vi "Pre Launch Init.vi"(11 "GlobalPlanner in":refnum<class "GlobalPlanner.lvclass"> caption="操作者输入") -> (0 "error out":errorcluster caption="错误输出", 3 "GlobalPlanner out":refnum<class "GlobalPlanner.lvclass"> caption="操作者输出")   [LabVIEW 2014, in "GlobalPlanner.lvlib" / "GlobalPlanner.lvclass"]
doc: "(<B>Filename</B>: Actor Framework.lvlib:Actor.lvclass:Pre Launch Init.vi)\n\nDefines behavior that occurs after the Launch Nested Actor method is invoked but before the actor's Actor Core method begins running.\n\nBy default, this method does nothing. A descendant class may override it to define behavior."
uses:
  GlobalPlanner.lvclass
  Global_var/Global_var.vi
  Wrapper_lib/zsActor/ActorWrapper.lvclass
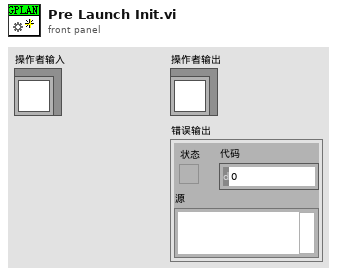
[diagram p1: front panel]
types:
  T1 = typedef "Point.ctl" = cluster{"x":dbl, "y":dbl, "z":dbl}
  T2 = typedef "P3AT_Current.ctl" = cluster{"max_vel":dbl, "max_rot":dbl, "now_pose_X":dbl, "now_pose_Y":dbl, "now_pose_Rot_deg":dbl, "Control_Mode":enum32{"Joy", "Map", "Voice", "Input", "Undefined"}}
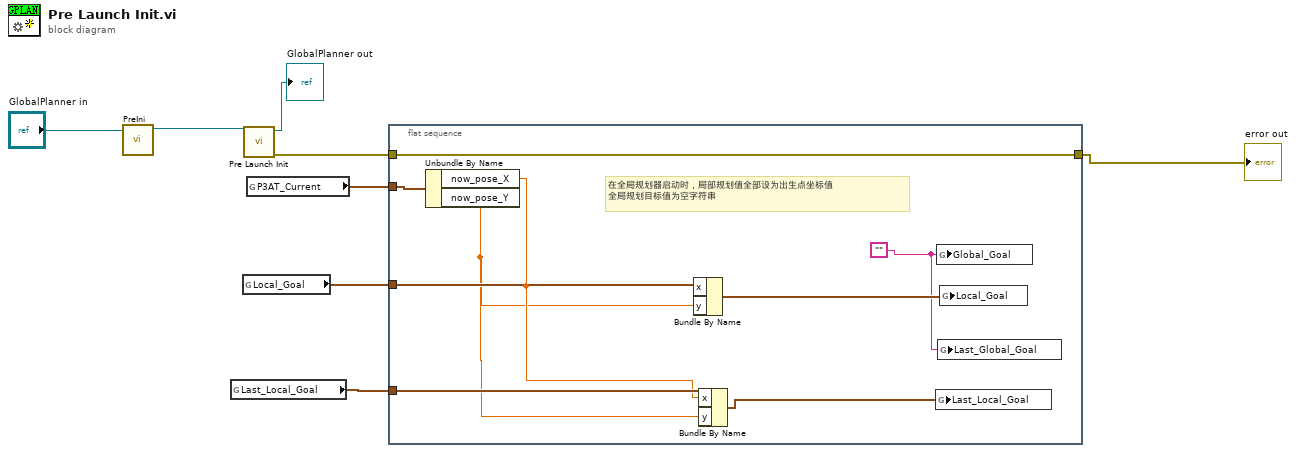
[diagram p0: block diagram]
diagram:
  n1 = call "PreIni.vi"("zsActor输入"="GlobalPlanner in") -> ("zsActor输出"=w1:refnum<class "GlobalPlanner.lvclass">)  [unwired: 9 in, 1 out]
  n2 = global read "Global_var.vi" "Last_Local_Goal"() -> (w3:T1)
  n3 = global read "Global_var.vi" "Local_Goal"() -> (w4:T1)
  n4 = call-parent "Pre Launch Init.vi"("Actor in"=w1) -> ("error out"=w7:errorcluster, "Actor out"=→"GlobalPlanner out":refnum<class "GlobalPlanner.lvclass">)  [unwired: 9 in]
  n5 = global read "Global_var.vi" "P3AT_Current"() -> (w5:T2)
  n6 = flat-sequence {
    tunnel: w7 -> [w17]
    tunnel: [w17] -> w6
    tunnel: w5 -> [w16]
    tunnel: w4 -> [w15]
    tunnel: w3 -> [w14]
    frame #0 {
      w9 = ""
      # "在全局规划器启动时，局部规划值全部设为出生点坐标值\n全局规划目标值为空字符串"
      n7 = Unbundle By Name(w16) -> ("now_pose_X"=w13:dbl, "now_pose_Y"=w12:dbl)
      n8 = Bundle By Name(cluster=w15, "x"=w13, "y"=w12) -> (w11:T1)
      n9 = Bundle By Name(cluster=w14, "x"=w13, "y"=w12) -> (w10:T1)
      n10 = global write "Global_var.vi" "Last_Local_Goal"(w10) -> ()
      n11 = global write "Global_var.vi" "Global_Goal"(w9) -> ()
      n12 = global write "Global_var.vi" "Last_Global_Goal"(w9) -> ()
      n13 = global write "Global_var.vi" "Local_Goal"(w11) -> ()
    }
  }
  "error out" <- w6
